vi "[ex ce] 5 Remote sound input & output.vi"() -> ()   [LabVIEW 2021]
doc: "<B>Remote sound input/output</B> (CE Client Example)\n\nThis example demonstartes how you can use CalcExpress for remote data acquisition and signal generation on example of sound input/output device. \n\nTo execute this example, you need run <B>\"[ex ce] CE Server Example.vi</B> on either local or remote computer. Also, you need a <B>sound card</B> on server side.\n\n::: CalcExpress Toolkit :::\nCopyright (c) 2000-2026 Konstantin Shifershteyn. All rights reserved."
panel:
  in  "To execute this example, you need run \"[ex ce] CE Server Example.vi\" on either local or remote computer. Also, you need a sound card on server side.\n-------------------------------------------\nThis example demonstrates how you can use CalcExpress for remote data acquisition and signal generation on example of sound wave device.":string="To execute this example, you need run \"[ex ce] CE Server Example.vi\" on either local or remote computer. Also, you need a sound card on server side.\n-------------------------------------------\nThis example demonstrates how you can use CalcExpress for remote data acquisition and signal generation on example of sound wave device. \n"
  out "vg led":bool
  out "so led":bool
  out "si led":bool
  out "vs led":bool
  in  "use TCP for local":bool
  in  "plot":u16(ring) caption="Select a variable from\nthe list to receive it\nfrom server and\nplot on graph" items=["-- plot var --", "in", "out"]
  in  "stop":bool
  in  "sndOut exp":string="out = in + 0.7 * shift(in, 5500);    // out = in + echo\nSndOut(SoundDevice, SoundRate, out); // play" caption="processing the input sound and playing the result on server's sound device"
  in  "sndIn exp":string="// read sound on server and save it in variable 'in' on server\nin = SndIn(SoundDevice, SoundRate, BufferSize);\n" caption="input sound from server's sound device"
  in  "SndOut":bool
  in  "SndIn":bool
  in  "var calc":bool
  in  "var exp":string="SoundDevice = 0;     // Sound Device number\nSoundRate   = 11025; // Sample Rate, Hz (11025/22050/44100)\nBufferSize  = 30000; // Buffer size, samples\na1dbl(\"in\"); a1dbl(\"out\"); // Input & Output sound buffers\n" caption="variables initializing"
  out "graph":dbl[](graph)
  in  "port":u32=3363
  in  "machine name (empty = local)":string
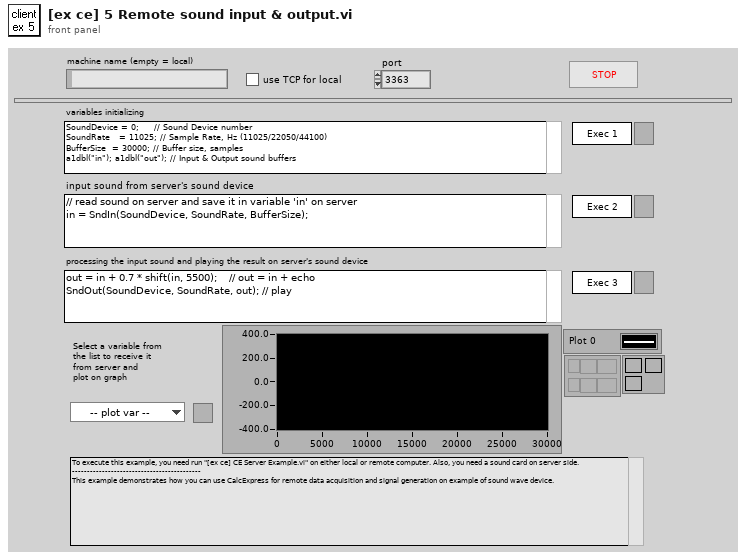
[diagram p1: front panel]
types:
  T1 = typedef "CE Session.ctl" = cluster{"VI refnum":refnum<vi>, "VC Handle":T2}
  T2 = typedef "VarMan Variable Context Handle.ctl" = i32
  T3 = typedef "CalcExpress Data Type.ctl" = enum32{"String", "DBL Number", "identifier", "1D Array of DBL", "2D Array of DBL", "CDB Number", "1D Array of CDB", "2D Array of CDB", "1D Array of String", "2D Array of String", "Unknown data type"}
  T4 = cluster{"type":T3, "dbl":dbl, "cdb":cdb, "str":string, "1d dbl":dbl[], "1d cdb":cdb[], "1d str":string[], "2d dbl":dbl[][], "2d cdb":cdb[][], "2d str":string[][]}
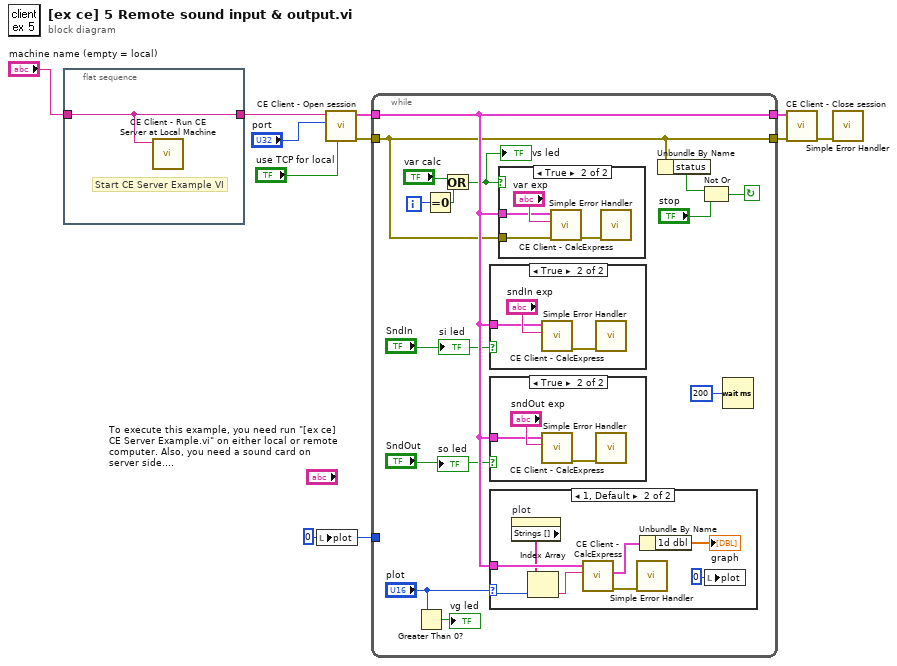
[diagram p0: block diagram]
diagram:
  w4 = u16 0
  n1 = flat-sequence {
    tunnel: [w11] -> w1
    tunnel: "machine name (empty = local)" -> [w11]
    frame #0 {
      # "Start CE Server Example VI"
      n2 = call "CE Client - Run CE Server at Local Machine.vi"("machine name"=w11) -> ()  [unwired: 9 in, 2 out]
    }
  }
  n3 = local write "plot"(w4) -> ()
  n4 = call "CE Client - Open session.vi"("use TCP for local (F)"="use TCP for local", "port number (3363)"="port", "machine name (empty - local)"=w1) -> ("error out"=w6:errorcluster, "CE session out"=w8:T1)  [unwired: 5 in]
  n5 = while {
    tunnel: w4 -> [_]
    tunnel: [w17] -> w5
    tunnel: w6 -> [w17]
    tunnel: [w19] -> w7
    tunnel: w8 -> [w19]
    i -> [w24]
    stop <- w20 continue-if-true
    n6 = Greater Than 0?(x="plot") -> (x > 0?=→"vg led":bool)
    n7 = Equal To 0?(x=w24) -> (x = 0?=w25:bool)
    n8 = Or(x="var calc", y=w25) -> (x .or. y?=w14:bool)
    "vs led" <- w14
    n9 = case shown="True" "SndIn" {
      tunnel: w19 -> [_ w37]
      frame False {
      }
      frame True {
        n10 = call "CE Client - CalcExpress.vi"("expression"="sndIn exp", "CE session"=w37) -> ("error out"=w39:errorcluster)  [unwired: 5 in, 2 out]
        n11 = call <vilib>:"Simple Error Handler.vi"("error in (no error)"=w39) -> ()  [unwired: 4 in, 5 out]
      }
    }
    n12 = case shown="True" "SndOut" {
      tunnel: w19 -> [_ w34]
      frame False {
      }
      frame True {
        n13 = call "CE Client - CalcExpress.vi"("expression"="sndOut exp", "CE session"=w34) -> ("error out"=w36:errorcluster)  [unwired: 5 in, 2 out]
        n14 = call <vilib>:"Simple Error Handler.vi"("error in (no error)"=w36) -> ()  [unwired: 4 in, 5 out]
      }
    }
    n15 = case shown="1, Default" "plot" {
      selector: "plot" -> [_ w30]
      tunnel: w19 -> [_ w32]
      frame 0 {
      }
      frame 1, Default {
        n16 = property on="plot" class="Ring (strict)"() -> ("Strings []"=w29:string[])  [unwired: 2 in, 2 out]
        n17 = Index Array(array=w29, index=w30) -> (element=w28:string)
        n18 = call "CE Client - CalcExpress.vi"("expression"=w28, "CE session"=w32) -> ("error out"=w33:errorcluster, "values out"=w26:T4)  [unwired: 5 in, 1 out]
        n19 = call <vilib>:"Simple Error Handler.vi"("error in (no error)"=w33) -> ()  [unwired: 4 in, 5 out]
        n20 = Unbundle By Name(w26) -> ("1d dbl"=→"graph":dbl[])
        n21 = local write "plot"(u16 0) -> ()
      }
    }
    n22 = case shown="True" w14 {
      tunnel: w19 -> [_ w41]
      tunnel: w17 -> [_ w40]
      frame False {
      }
      frame True {
        n23 = call "CE Client - CalcExpress.vi"("error in"=w40, "expression"="var exp", "CE session"=w41) -> ("error out"=w42:errorcluster)  [unwired: 4 in, 2 out]
        n24 = call <vilib>:"Simple Error Handler.vi"("error in (no error)"=w42) -> ()  [unwired: 4 in, 5 out]
      }
    }
    n25 = Unbundle By Name(w17) -> ("status"=w22:bool)
    n26 = Not Or(1:"stop", 2:w22) -> (0:w20:bool)
    n27 = Wait (ms)(milliseconds to wait=u32 200) -> ()  [unwired: 1 out]
    "si led" <- "SndIn"
    "so led" <- "SndOut"
  }
  n28 = call "CE Client - Close session.vi"("error in"=w5, "CE session"=w7) -> ("error out"=w9:errorcluster)  [unwired: 6 in, 1 out]
  n29 = call <vilib>:"Simple Error Handler.vi"("error in (no error)"=w9) -> ()  [unwired: 4 in, 5 out]
